vi "HostMem Empty.vi"(8 "error in (no error)":errorcluster, 11 "HostMem in":refnum<class "HostMem.lvclass">) -> (0 "error out":errorcluster, 2 "IsEmpty":bool, 3 "HostMem out":refnum<class "HostMem.lvclass">)   [LabVIEW 2020, in "OpenLvVision_OpenCv.lvlib" / "Cuda.lvlib" / "HostMem.lvclass"]
doc: "Returns true if the HostMem object has no allocated data or a size of zero."
uses:
  HostMem.lvclass
  C:/Users/lukas/Downloads/OpenLvVision_OpenCv/SourceCode/LabView/OpenLvVision_OpenCv/_LvHelpers/EdvrObject/EdvrObject.lvclass
  _LvHelpers/EdvrObject/EdvrObject.lvclass/EdvrObject.ctl
  OpenLvVision_OpenCv.lvlib
  <vilib>/Utility/error.llb/Error Cluster From Error Code.vi
  <vilib>/ErrorRing/Error Ring.xnode
  _LvHelpers/EdvrObject/EdvrObject.lvclass
  Dlls/OlvOpenCvWrapper.dll
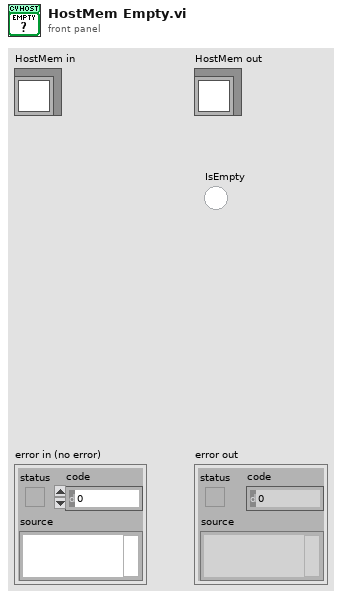
[diagram p1: front panel]
types:
  T1 = typedef "OpenLvVision_OpenCv.lvlib/EdvrObject.lvclass/Edvr.ctl" = refnum<data-value>
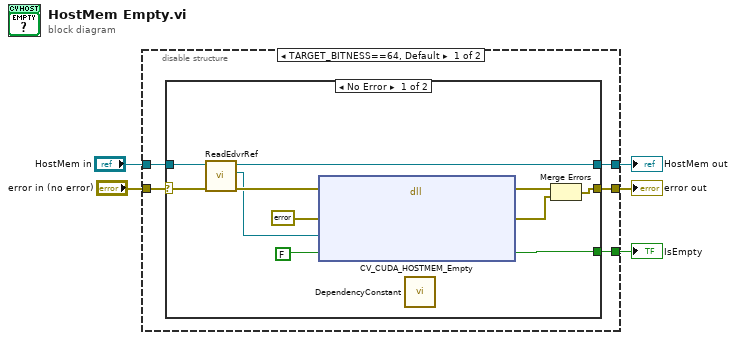
[diagram p0: block diagram]
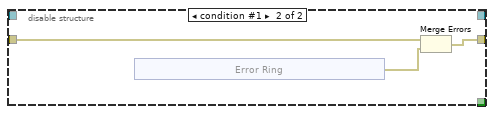
[diagram p3: hidden frame]
diagram:
  n1 = disable-structure shown="TARGET_BITNESS==64, Default" {
    disable-tunnel: "error in (no error)" -> [w10 w25]
    disable-tunnel: [w9 w26] -> w4
    disable-tunnel: "HostMem in" -> [w8 _]
    disable-tunnel: [w7 _] -> w2
    disable-tunnel: [w6 _] -> w1
    frame condition #0 (active) {
      n2 = case shown="No Error" w10 {
        selector: w10 -> [w18 w23]
        tunnel: [w13 w23] -> w9
        tunnel: w8 -> [w17 w22]
        tunnel: [w14 w22] -> w7
        tunnel: [w12 _] -> w6
        frame No Error {
          n3 = call "ReadEdvrRef.vi"("error in (no error)"=w18, "EdvrObject in"=w17) -> ("error out"=w16:errorcluster, "Edvr"=w15:T1, "EdvrObject out"=w14:refnum<class "HostMem.lvclass">)  [unwired: 7 in]
          n4 = dll-call lib="C:/Users/lukas/Downloads/OpenLvVision_OpenCv/SourceCode/LabView/OpenLvVision_OpenCv/Dlls/OlvOpenCvWrapper.dll" fn="CV_CUDA_HOSTMEM_Empty"(error in=w16, "Error"=errorcluster {"status"=FALSE, "code"=0, "source"=""} ("error out"), "edvrRef"=w15, "result"=FALSE) -> (error out=w21:errorcluster, "Error"=w20:errorcluster, "result"=w12:bool)  [unwired: 4 in, 1 out]
          n5 = call "DependencyConstant.vi"() -> ()  [unwired: 12 in]
          n6 = Merge Errors(w21, w20) -> (w13:errorcluster)
        }
        frame Error {
        }
      }
    }
    frame condition #1 {
      n7 = xnode "Error Ring"() -> ("error out"=w24:errorcluster)
      n8 = Merge Errors(w25, w24) -> (w26:errorcluster)
    }
  }
  "error out" <- w4
  "HostMem out" <- w2
  "IsEmpty" <- w1
